vi "PostMessageW Wrapper Template.vi"(0 "hWnd":u64, 5 "Msg":u32, 7 "wParam":u64, 9 "lParam":i64, 11 "error in (no error)":errorcluster) -> (4 "return value":i32, 15 "error out":errorcluster)   [LabVIEW 2020]
doc: "Posts a message to the message queue of the window hWnd through user32.dll PostMessageW (stdcall, called in any thread) and returns without waiting for it to be processed. return value is the Win32 BOOL: non-zero on success, 0 on failure (call GetLastError for the reason). When error in carries an error the DLL is not called. Generated by tools\\Build Win32 Wrappers.vi - do not edit by hand, rebuild it."
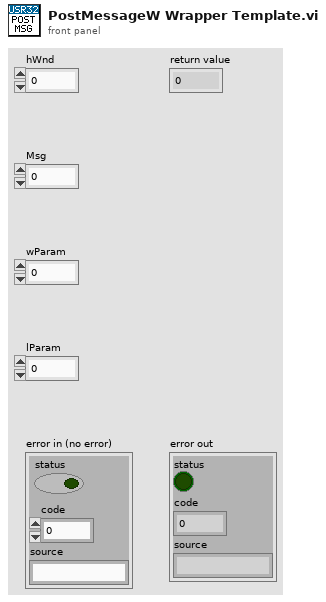
[diagram p1: front panel]
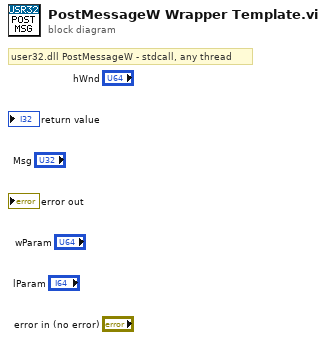
[diagram p0: block diagram]
diagram:
  # "user32.dll PostMessageW - stdcall, any thread"
